vi "RemoteVI Fixture Mods.vi"(0 "PlatMods":T1, 11 "error in":errorcluster) -> (4 "mods":string, 15 "error out":errorcluster)   [LabVIEW 2020]
doc: "Event-log helper of RemoteVI Fixture.vi. Turns an event's PlatMods cluster into the log's modifier field: S for Shift, C for Ctrl, A for Alt, in that order, or - when none is held. error in is passed through unchanged."
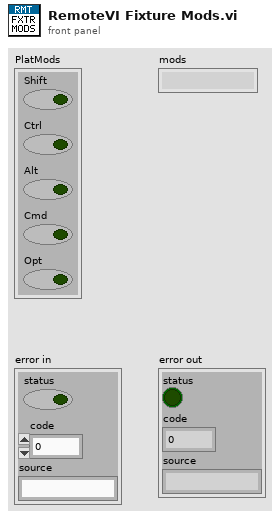
[diagram p1: front panel]
types:
  T1 = cluster{"Shift":bool, "Ctrl":bool, "Alt":bool, "Cmd":bool, "Opt":bool}
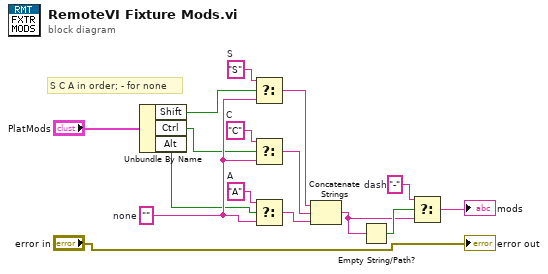
[diagram p0: block diagram]
diagram:
  w10 = "-"  # dash
  w9 = ""  # none
  w8 = "A"  # A
  w7 = "C"  # C
  w6 = "S"  # S
  # "S C A in order; - for none"
  n1 = Unbundle By Name("PlatMods") -> ("Shift"=w3:bool, "Ctrl"=w4:bool, "Alt"=w5:bool)
  n2 = Select(t=w6, s=w3, f=w9) -> (s? t:f=w11:string)
  n3 = Select(t=w7, s=w4, f=w9) -> (s? t:f=w12:string)
  n4 = Select(t=w8, s=w5, f=w9) -> (s? t:f=w13:string)
  n5 = Concatenate Strings(w11, w12, w13) -> (w14:string)
  n6 = Empty String/Path?(string/path=w14) -> (empty?=w15:bool)
  n7 = Select(t=w10, s=w15, f=w14) -> (s? t:f=→"mods":string)
  "error out" <- "error in"
